vi "start SA Measurement with OPC for single sweep.vi"(8 "error in (no error)":errorcluster, 9 "with OPC?":bool, 11 "Keysight 9020A in":refnum<class "Keysight 9020A.lvclass">) -> (0 "error out":errorcluster, 3 "Keysight 9020A out":refnum<class "Keysight 9020A.lvclass">)   [LabVIEW 2023, in "Spectrum Analyzer.lvlib" / "Keysight 9020A.lvclass"]
uses:
  Keysight 9020A.lvclass
  Keysight 9020A.lvclass/Keysight 9020A.ctl
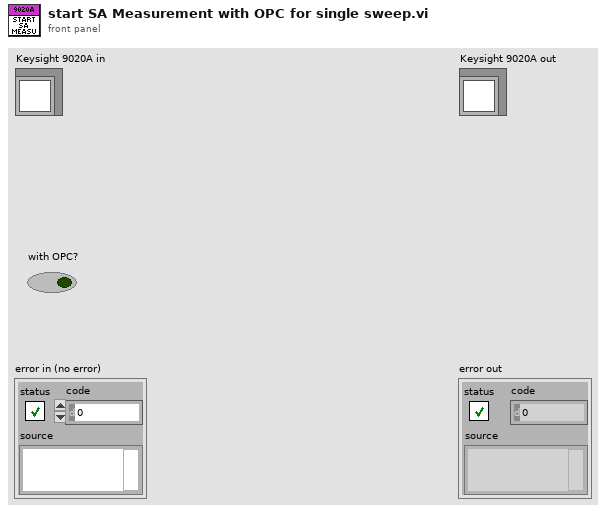
[diagram p1: front panel]
types:
  T1 = typedef "Spectrum Analyzer.lvlib/TYPE Measurement Preset.ctl" = enum16{"Sweep SA Mode", "Channel Power", "Occupied BW", "ACP", "Spurious Emission", "Spurious Emission Mask", "Burst Power (Transmit Power)"}
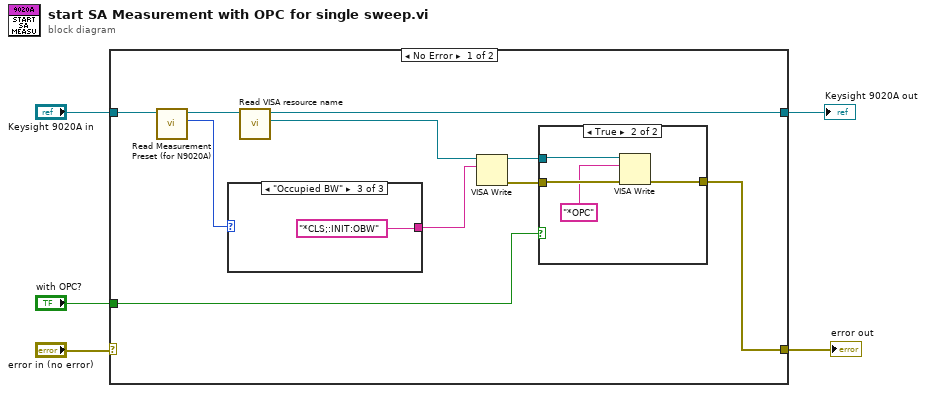
[diagram p0: block diagram]
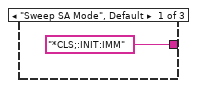
[diagram p3: hidden frame]
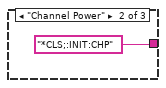
[diagram p4: hidden frame]
diagram:
  n1 = case shown="No Error" "error in (no error)" {
    selector: "error in (no error)" -> [_ w24]
    tunnel: "Keysight 9020A in" -> [w8 w25]
    tunnel: [w15 w25] -> w4
    tunnel: [w9 w24] -> w1
    tunnel: "with OPC?" -> [w11 _]
    frame No Error {
      n2 = call "Read Measurement Preset (for N9020A).vi"("Keysight 9020A in"=w8) -> ("Measurement Preset"=w6:T1, "Keysight 9020A out"=w7:refnum<class "Keysight 9020A.lvclass">)  [unwired: 8 in, 1 out]
      n3 = case shown="\"Occupied BW\"" w6 {
        tunnel: ["*CLS;:INIT:IMM" ("write buffer") "*CLS;:INIT:CHP" ("write buffer") "*CLS;:INIT:OBW" ("write buffer")] -> w13
        frame "Sweep SA Mode", Default {
        }
        frame "Channel Power" {
        }
        frame "Occupied BW" {
        }
      }
      n4 = call "Read VISA resource name.vi"("Keysight 9020A in"=w7) -> ("VISA resource name"=w14:refnum<visa-resource-name>, "Keysight 9020A out"=w15:refnum<class "Keysight 9020A.lvclass">)  [unwired: 8 in, 1 out]
      n5 = VISA Write(VISA resource name=w14, write buffer=w13) -> (VISA resource name out=w12:refnum<visa-resource-name>, error out=w10:errorcluster)  [unwired: 1 in, 1 out]
      n6 = case shown="True" w11 {
        tunnel: w12 -> [_ w20]
        tunnel: w10 -> [w16 w19]
        tunnel: [w16 w18] -> w9
        frame False {
        }
        frame True {
          n7 = VISA Write(VISA resource name=w20, write buffer="*OPC", error in (no error)=w19) -> (error out=w18:errorcluster)  [unwired: 2 out]
        }
      }
    }
    frame Error {
    }
  }
  "error out" <- w1
  "Keysight 9020A out" <- w4
